vi "Voltage calibration.vi"(11 "INPUT VOLTAGE":dbl) -> (3 "voltage output":dbl)   [LabVIEW 2026]
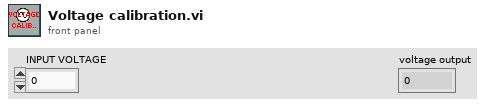
[diagram p1: front panel]
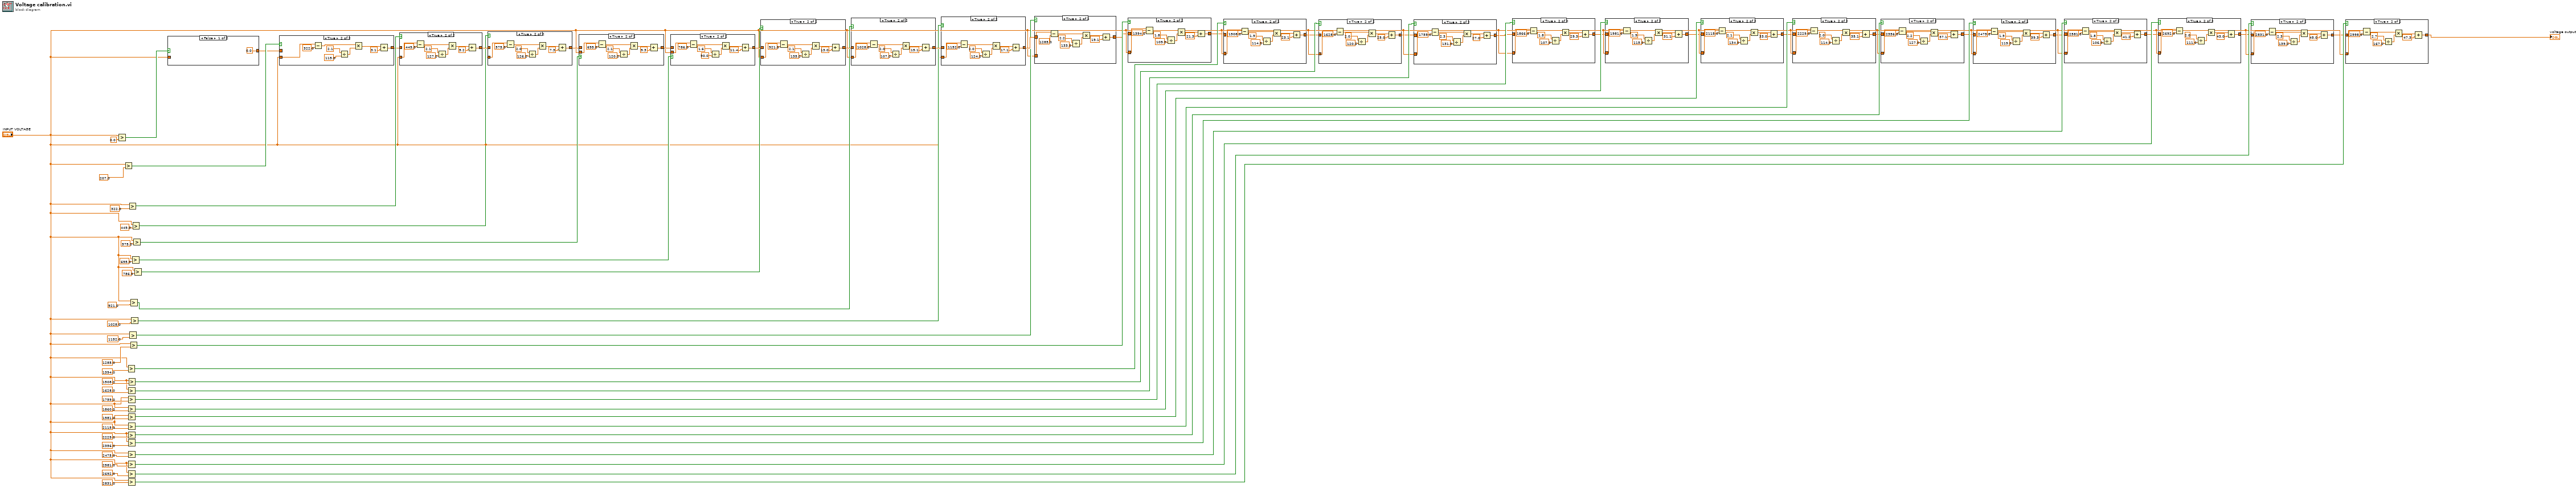
[diagram p0: block diagram]
diagram:
  n1 = Greater?(x="INPUT VOLTAGE", y=0.0) -> (0:w73:bool)
  n2 = Greater?(x="INPUT VOLTAGE", y=207.0) -> (0:w70:bool)
  n3 = Greater?(x="INPUT VOLTAGE", y=1394.0) -> (0:w29:bool)
  n4 = Greater?(x="INPUT VOLTAGE", y=1628.0) -> (0:w27:bool)
  n5 = Greater?(x="INPUT VOLTAGE", y=1759.0) -> (0:w26:bool)
  n6 = Greater?(x="INPUT VOLTAGE", y=1860.0) -> (0:w25:bool)
  n7 = Greater?(x="INPUT VOLTAGE", y=1981.0) -> (0:w24:bool)
  n8 = Greater?(x="INPUT VOLTAGE", y=2115.0) -> (0:w23:bool)
  n9 = Greater?(x="INPUT VOLTAGE", y=2229.0) -> (0:w22:bool)
  n10 = Greater?(x="INPUT VOLTAGE", y=2356.0) -> (0:w21:bool)
  n11 = Greater?(x="INPUT VOLTAGE", y=2475.0) -> (0:w20:bool)
  n12 = Greater?(x="INPUT VOLTAGE", y=2581.0) -> (0:w19:bool)
  n13 = Greater?(x="INPUT VOLTAGE", y=2692.0) -> (0:w18:bool)
  n14 = Greater?(x="INPUT VOLTAGE", y=2831.0) -> (0:w17:bool)
  n15 = Greater?(x="INPUT VOLTAGE", y=1508.0) -> (0:w28:bool)
  n16 = Greater?(x="INPUT VOLTAGE", y=322.0) -> (0:w68:bool)
  n17 = Greater?(x="INPUT VOLTAGE", y=1152.0) -> (0:w46:bool)
  n18 = Greater?(x="INPUT VOLTAGE", y=1285.0) -> (0:w44:bool)
  n19 = Greater?(x="INPUT VOLTAGE", y=921.0) -> (0:w51:bool)
  n20 = Greater?(x="INPUT VOLTAGE", y=1028.0) -> (0:w47:bool)
  n21 = Greater?(x="INPUT VOLTAGE", y=695.0) -> (0:w59:bool)
  n22 = Greater?(x="INPUT VOLTAGE", y=449.0) -> (0:w65:bool)
  n23 = Greater?(x="INPUT VOLTAGE", y=575.0) -> (0:w61:bool)
  n24 = Greater?(x="INPUT VOLTAGE", y=786.0) -> (0:w55:bool)
  n25 = case shown="False" w73 {
    tunnel: [0.0 ("y") w77] -> w53
    tunnel: "INPUT VOLTAGE" -> [_ w78]
    frame False {
    }
    frame True {
      n26 = Divide(x=3.1 ("y"), y=207.0) -> (x/y=w81:dbl)
      n27 = Multiply(x=w81, y=w78) -> (x*y=w75:dbl)
      n28 = Add(x=w75, y=0.0 ("x")) -> (x+y=w77:dbl)
    }
  }
  n29 = case shown="True" w70 {
    tunnel: w53 -> [w82 _]
    tunnel: [w82 w91] -> w67
    tunnel: "INPUT VOLTAGE" -> [_ w88]
    frame False {
    }
    frame True {
      n30 = Subtract(x=w88, y=322.0) -> (x-y=w85:dbl)
      n31 = Divide(x=2.1, y=115.0) -> (x/y=w84:dbl)
      n32 = Multiply(x=w85, y=w84) -> (x*y=w83:dbl)
      n33 = Add(x=w83, y=3.1) -> (x+y=w91:dbl)
    }
  }
  n34 = case shown="True" w68 {
    tunnel: [w92 w100] -> w66
    tunnel: w67 -> [w92 _]
    tunnel: "INPUT VOLTAGE" -> [_ w98]
    frame False {
    }
    frame True {
      n35 = Subtract(x=w98, y=449.0) -> (x-y=w95:dbl)
      n36 = Divide(x=2.1, y=127.0) -> (x/y=w94:dbl)
      n37 = Multiply(x=w95, y=w94) -> (x*y=w93:dbl)
      n38 = Add(x=w93, y=5.2) -> (x+y=w100:dbl)
    }
  }
  n39 = case shown="True" w65 {
    tunnel: w66 -> [w102 _]
    tunnel: "INPUT VOLTAGE" -> [_ w110]
    tunnel: [w102 w108] -> w62
    frame False {
    }
    frame True {
      n40 = Subtract(x=w110, y=575.0) -> (x-y=w105:dbl)
      n41 = Divide(x=2.0, y=126.0) -> (x/y=w104:dbl)
      n42 = Multiply(x=w105, y=w104) -> (x*y=w103:dbl)
      n43 = Add(x=w103, y=7.3) -> (x+y=w108:dbl)
    }
  }
  n44 = case shown="True" w61 {
    tunnel: [w112 w118] -> w58
    tunnel: w62 -> [w112 _]
    tunnel: "INPUT VOLTAGE" -> [_ w120]
    frame False {
    }
    frame True {
      n45 = Subtract(x=w120, y=695.0) -> (x-y=w114:dbl)
      n46 = Divide(x=2.1, y=120.0) -> (x/y=w116:dbl)
      n47 = Multiply(x=w114, y=w116) -> (x*y=w113:dbl)
      n48 = Add(x=w113, y=9.3) -> (x+y=w118:dbl)
    }
  }
  n49 = case shown="True" w59 {
    tunnel: [w122 w128] -> w56
    tunnel: w58 -> [w122 _]
    tunnel: "INPUT VOLTAGE" -> [_ w131]
    frame False {
    }
    frame True {
      n50 = Subtract(x=w131, y=786.0) -> (x-y=w124:dbl)
      n51 = Divide(x=1.6, y=90.0) -> (x/y=w125:dbl)
      n52 = Multiply(x=w124, y=w125) -> (x*y=w123:dbl)
      n53 = Add(x=w123, y=11.4) -> (x+y=w128:dbl)
    }
  }
  n54 = case shown="True" w55 {
    tunnel: [w132 w138] -> w54
    tunnel: "INPUT VOLTAGE" -> [_ w139]
    tunnel: w56 -> [w132 _]
    frame False {
    }
    frame True {
      n55 = Subtract(x=w139, y=921.0) -> (x-y=w134:dbl)
      n56 = Divide(x=2.1, y=135.0) -> (x/y=w135:dbl)
      n57 = Multiply(x=w134, y=w135) -> (x*y=w133:dbl)
      n58 = Add(x=w133, y=13.0) -> (x+y=w138:dbl)
    }
  }
  n59 = case shown="True" w51 {
    tunnel: [w142 w147] -> w50
    tunnel: w54 -> [w142 _]
    tunnel: "INPUT VOLTAGE" -> [_ w149]
    frame False {
    }
    frame True {
      n60 = Subtract(x=w149, y=1028.0) -> (x-y=w144:dbl)
      n61 = Divide(x=2.0, y=107.0) -> (x/y=w143:dbl)
      n62 = Multiply(x=w144, y=w143) -> (x*y=w145:dbl)
      n63 = Add(x=w145, y=15.1) -> (x+y=w147:dbl)
    }
  }
  n64 = case shown="True" w47 {
    tunnel: [w152 w157] -> w49
    tunnel: w50 -> [w152 _]
    tunnel: "INPUT VOLTAGE" -> [_ w160]
    frame False {
    }
    frame True {
      n65 = Subtract(x=w160, y=1152.0) -> (x-y=w156:dbl)
      n66 = Divide(x=2.0, y=124.0) -> (x/y=w155:dbl)
      n67 = Multiply(x=w156, y=w155) -> (x*y=w153:dbl)
      n68 = Add(x=w153, y=17.1) -> (x+y=w157:dbl)
    }
  }
  n69 = case shown="True" w46 {
    tunnel: [w162 w167] -> w15
    tunnel: w49 -> [w162 _]
    tunnel: "INPUT VOLTAGE" -> [_ w169]
    frame False {
    }
    frame True {
      n70 = Subtract(x=w169, y=1285.0) -> (x-y=w165:dbl)
      n71 = Divide(x=2.2, y=133.0) -> (x/y=w164:dbl)
      n72 = Multiply(x=w165, y=w164) -> (x*y=w163:dbl)
      n73 = Add(x=w163, y=19.1) -> (x+y=w167:dbl)
    }
  }
  n74 = case shown="True" w44 {
    tunnel: [w172 w177] -> w14
    tunnel: w15 -> [w172 _]
    tunnel: "INPUT VOLTAGE" -> [_ w179]
    frame False {
    }
    frame True {
      n75 = Subtract(x=w179, y=1394.0) -> (x-y=w175:dbl)
      n76 = Divide(x=1.8, y=109.0) -> (x/y=w174:dbl)
      n77 = Multiply(x=w175, y=w174) -> (x*y=w173:dbl)
      n78 = Add(x=w173, y=21.3) -> (x+y=w177:dbl)
    }
  }
  n79 = case shown="True" w29 {
    tunnel: [w182 w187] -> w13
    tunnel: w14 -> [w182 _]
    tunnel: "INPUT VOLTAGE" -> [_ w189]
    frame False {
    }
    frame True {
      n80 = Subtract(x=w189, y=1508.0) -> (x-y=w185:dbl)
      n81 = Divide(x=1.9, y=114.0) -> (x/y=w184:dbl)
      n82 = Multiply(x=w185, y=w184) -> (x*y=w183:dbl)
      n83 = Add(x=w183, y=23.1) -> (x+y=w187:dbl)
    }
  }
  n84 = case shown="True" w28 {
    tunnel: [w192 w197] -> w12
    tunnel: w13 -> [w192 _]
    tunnel: "INPUT VOLTAGE" -> [_ w199]
    frame False {
    }
    frame True {
      n85 = Subtract(x=w199, y=1628.0) -> (x-y=w195:dbl)
      n86 = Divide(x=2.0, y=120.0) -> (x/y=w194:dbl)
      n87 = Multiply(x=w195, y=w194) -> (x*y=w193:dbl)
      n88 = Add(x=w193, y=25.0) -> (x+y=w197:dbl)
    }
  }
  n89 = case shown="True" w27 {
    tunnel: [w202 w207] -> w11
    tunnel: w12 -> [w202 _]
    tunnel: "INPUT VOLTAGE" -> [_ w209]
    frame False {
    }
    frame True {
      n90 = Subtract(x=w209, y=1759.0) -> (x-y=w205:dbl)
      n91 = Divide(x=2.3, y=131.0) -> (x/y=w204:dbl)
      n92 = Multiply(x=w205, y=w204) -> (x*y=w203:dbl)
      n93 = Add(x=w203, y=27.0) -> (x+y=w207:dbl)
    }
  }
  n94 = case shown="True" w26 {
    tunnel: [w212 w217] -> w10
    tunnel: w11 -> [w212 _]
    tunnel: "INPUT VOLTAGE" -> [_ w219]
    frame False {
    }
    frame True {
      n95 = Subtract(x=w219, y=1866.0) -> (x-y=w215:dbl)
      n96 = Divide(x=1.8, y=107.0) -> (x/y=w214:dbl)
      n97 = Multiply(x=w215, y=w214) -> (x*y=w213:dbl)
      n98 = Add(x=w213, y=29.3) -> (x+y=w217:dbl)
    }
  }
  n99 = case shown="True" w25 {
    tunnel: [w222 w227] -> w9
    tunnel: w10 -> [w222 _]
    tunnel: "INPUT VOLTAGE" -> [_ w229]
    frame False {
    }
    frame True {
      n100 = Subtract(x=w229, y=1981.0) -> (x-y=w225:dbl)
      n101 = Divide(x=1.9, y=115.0) -> (x/y=w224:dbl)
      n102 = Multiply(x=w225, y=w224) -> (x*y=w223:dbl)
      n103 = Add(x=w223, y=31.1) -> (x+y=w227:dbl)
    }
  }
  n104 = case shown="True" w24 {
    tunnel: [w232 w237] -> w8
    tunnel: w9 -> [w232 _]
    tunnel: "INPUT VOLTAGE" -> [_ w239]
    frame False {
    }
    frame True {
      n105 = Subtract(x=w239, y=2115.0) -> (x-y=w235:dbl)
      n106 = Divide(x=2.1, y=134.0) -> (x/y=w234:dbl)
      n107 = Multiply(x=w235, y=w234) -> (x*y=w233:dbl)
      n108 = Add(x=w233, y=33.0) -> (x+y=w237:dbl)
    }
  }
  n109 = case shown="True" w23 {
    tunnel: [w242 w247] -> w7
    tunnel: w8 -> [w242 _]
    tunnel: "INPUT VOLTAGE" -> [_ w249]
    frame False {
    }
    frame True {
      n110 = Subtract(x=w249, y=2229.0) -> (x-y=w245:dbl)
      n111 = Divide(x=2.0, y=114.0) -> (x/y=w244:dbl)
      n112 = Multiply(x=w245, y=w244) -> (x*y=w243:dbl)
      n113 = Add(x=w243, y=35.1) -> (x+y=w247:dbl)
    }
  }
  n114 = case shown="True" w22 {
    tunnel: [w252 w257] -> w6
    tunnel: w7 -> [w252 _]
    tunnel: "INPUT VOLTAGE" -> [_ w259]
    frame False {
    }
    frame True {
      n115 = Subtract(x=w259, y=2356.0) -> (x-y=w255:dbl)
      n116 = Divide(x=2.2, y=127.0) -> (x/y=w254:dbl)
      n117 = Multiply(x=w255, y=w254) -> (x*y=w253:dbl)
      n118 = Add(x=w253, y=37.1) -> (x+y=w257:dbl)
    }
  }
  n119 = case shown="True" w21 {
    tunnel: [w262 w267] -> w5
    tunnel: w6 -> [w262 _]
    tunnel: "INPUT VOLTAGE" -> [_ w269]
    frame False {
    }
    frame True {
      n120 = Subtract(x=w269, y=2475.0) -> (x-y=w265:dbl)
      n121 = Divide(x=1.9, y=119.0) -> (x/y=w264:dbl)
      n122 = Multiply(x=w265, y=w264) -> (x*y=w263:dbl)
      n123 = Add(x=w263, y=39.3) -> (x+y=w267:dbl)
    }
  }
  n124 = case shown="True" w20 {
    tunnel: [w272 w277] -> w4
    tunnel: w5 -> [w272 _]
    tunnel: "INPUT VOLTAGE" -> [_ w279]
    frame False {
    }
    frame True {
      n125 = Subtract(x=w279, y=2581.0) -> (x-y=w275:dbl)
      n126 = Divide(x=1.8, y=106.0) -> (x/y=w274:dbl)
      n127 = Multiply(x=w275, y=w274) -> (x*y=w273:dbl)
      n128 = Add(x=w273, y=41.2) -> (x+y=w277:dbl)
    }
  }
  n129 = case shown="True" w19 {
    tunnel: [w282 w287] -> w3
    tunnel: w4 -> [w282 _]
    tunnel: "INPUT VOLTAGE" -> [_ w289]
    frame False {
    }
    frame True {
      n130 = Subtract(x=w289, y=2692.0) -> (x-y=w285:dbl)
      n131 = Divide(x=2.0, y=111.0) -> (x/y=w284:dbl)
      n132 = Multiply(x=w285, y=w284) -> (x*y=w283:dbl)
      n133 = Add(x=w283, y=43.0) -> (x+y=w287:dbl)
    }
  }
  n134 = case shown="True" w18 {
    tunnel: [w292 w297] -> w2
    tunnel: w3 -> [w292 _]
    tunnel: "INPUT VOLTAGE" -> [_ w299]
    frame False {
    }
    frame True {
      n135 = Subtract(x=w299, y=2831.0) -> (x-y=w295:dbl)
      n136 = Divide(x=2.3, y=139.0) -> (x/y=w294:dbl)
      n137 = Multiply(x=w295, y=w294) -> (x*y=w293:dbl)
      n138 = Add(x=w293, y=45.0) -> (x+y=w297:dbl)
    }
  }
  n139 = case shown="True" w17 {
    tunnel: [w302 w307] -> w1
    tunnel: w2 -> [w302 _]
    tunnel: "INPUT VOLTAGE" -> [_ w309]
    frame False {
    }
    frame True {
      n140 = Subtract(x=w309, y=2998.0) -> (x-y=w305:dbl)
      n141 = Divide(x=2.7, y=167.0) -> (x/y=w304:dbl)
      n142 = Multiply(x=w305, y=w304) -> (x*y=w303:dbl)
      n143 = Add(x=w303, y=47.3) -> (x+y=w307:dbl)
    }
  }
  "voltage output" <- w1
